vi "load asynchronous call.vi"   [LabVIEW 2013, in "NISE Tools Drop Templates.lvlib"]
uses:
  NISE Tools Drop Templates.lvlib
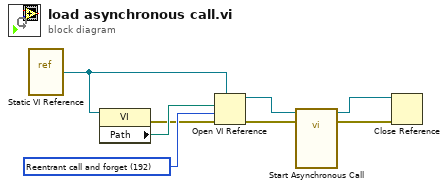
[diagram p0: block diagram]
diagram:
  w8 = 192 items=["Prepare to call and forget"=128, "Prepare to call and collect"=256, "Reentrant call and forget"=192, "Reentrant call and collect"=320] ("VI Server Options")
  n1 = vi-ref "Static VI Reference"() -> ("vi reference"=w1:refnum<vi>)
  n2 = property class="VI"(reference=w1) -> (error out=w6:errorcluster, "Path"=w7:path)  [unwired: 1 in, 1 out]
  n3 = Open VI Reference(type specifier VI Refnum (for type only)=w1, vi path=w7, options=w8, error in (no error)=w6) -> (vi reference=w4:refnum<vi>, error out=w5:errorcluster)  [unwired: 2 in]
  n4 = call-by-ref "Start Asynchronous Call"(reference=w4, error in=w5) -> (reference out=w2:refnum<vi>, error out=w3:errorcluster)  [unwired: 12 in]
  n5 = Close Reference(reference=w2, error in (no error)=w3) -> ()  [unwired: 1 out]
